vi "Link Test Channels.vi"(7 "gRPC ID in":T4, 8 "error in (no error)":errorcluster, 10 "Channels":T1[](array[typedef]), 11 "CIFCorePlugin in":refnum<class "CIFCorePlugin.lvclass">) -> (0 "error out":errorcluster, 3 "CIFCorePlugin out":refnum<class "CIFCorePlugin.lvclass">)   [LabVIEW 2021, in "CAN_Writer_NIXNET_Test_Helpers.lvlib"]
uses:
  CAN_Writer_NIXNET_Test_Helpers.lvlib
  <vilib>/CIF Foundation/CIF Core/CIFCore/Grpc/CIFCoreWrapper/CIFCoreWrapper.lvlib
  <vilib>/CIF Foundation/CIF Channels Core/ChannelCommon/ChannelCommon.lvlib
  <vilib>/CIF Foundation/CIF Channels Core/ChannelCommon/typedef/New FIFO Instance Configuration.ctl
  <vilib>/CIF Foundation/CIF Channels Core/CIFChannels/CIFChannels.lvclass
  <vilib>/CIF Foundation/CIF Core/CIFCore/Common/Typedef/FIFO Publisher.ctl
  <vilib>/CIF Foundation/CIF Core/CIFCore/Common/CIFCoreCommon.lvlib
  <vilib>/CIF Foundation/CIF Core/CIFCore/Grpc/CIFCoreChannel_client/RPC Messages/cif_channelcore_SetConnectionRequest.ctl
  <vilib>/CIF Foundation/CIF Core/CIFCore/Grpc/CIFCoreChannel_client/CIFCoreChannel_client.lvlib
  <vilib>/CIF Foundation/CIF Core/CIFCore/Class/CIFCorePlugin.lvclass
  <vilib>/gRPC/LabVIEW gRPC Library/Shared/grpcId.ctl
  <vilib>/gRPC/LabVIEW gRPC Library/grpc-lvsupport-release.lvlib
  <vilib>/CIF Foundation/CIF Core/CIFCore/Grpc/CIFCorePlugin_client/RPC Messages/cif_management_common_ChannelPattern.ctl
  <vilib>/CIF Foundation/CIF Core/CIFCore/Grpc/CIFCorePlugin_client/CIFCorePlugin_client.lvlib
  <vilib>/CIF Foundation/CIF Core/CIFCore/Grpc/CIFCorePlugin_client/RPC Messages/cif_management_common_ChannelDirection.ctl
  <vilib>/CIF Foundation/CIF Core/CIFCore/Grpc/CIFCorePlugin_client/RPC Messages/cif_management_common_Channel.ctl
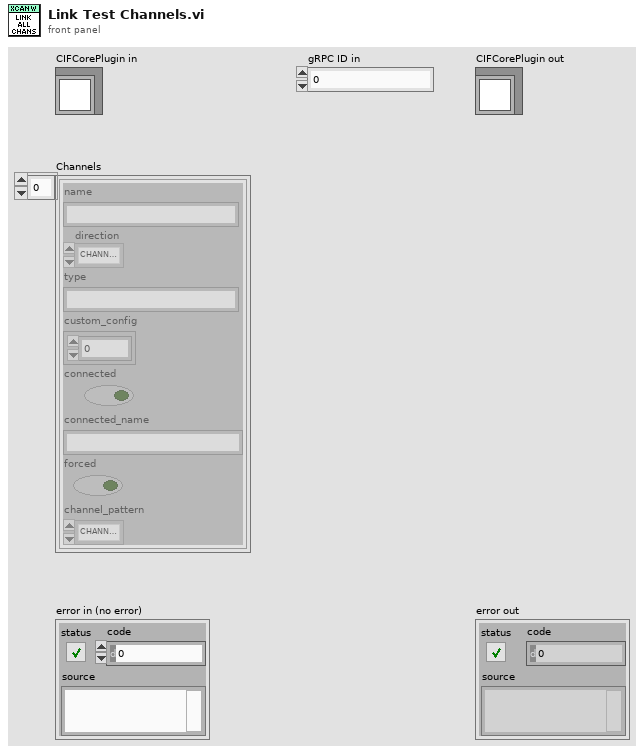
[diagram p1: front panel]
types:
  T1 = typedef "CIFCorePlugin_client.lvlib/cif_management_common_Channel.ctl" = cluster{"name":string, "direction":T2, "type":string, "custom_config":u8[], "connected":bool, "connected_name":string, "forced":bool, "channel_pattern":T3}
  T2 = typedef "CIFCorePlugin_client.lvlib/cif_management_common_ChannelDirection.ctl" = enum32{"CHANNELDIRECTION_UNKNOWN", "CHANNELDIRECTION_PUBLISHER", "CHANNELDIRECTION_SUBSCRIBER"}
  T3 = typedef "CIFCorePlugin_client.lvlib/cif_management_common_ChannelPattern.ctl" = enum32{"CHANNELPATTERN_UNKNOWN", "CHANNELPATTERN_TAG", "CHANNELPATTERN_FIFO", "CHANNELPATTERN_MULTIFIFO", "CHANNELPATTERN_BACKPRESSUREFIFO"}
  T4 = typedef "grpc-lvsupport-release.lvlib/grpcId.ctl" = u64
  T5 = typedef "ChannelCommon.lvlib/New FIFO Instance Configuration.ctl" = cluster{"Backpressure":bool, "Bytes/Message Override":u32, "Messages/FIFO Override":u32, "Custom Data":u8[]}
  T6 = typedef "CIFCoreCommon.lvlib/FIFO Publisher.ctl" = cluster{"Publisher Name":string, "New FIFO Instance Config":T5}
  T7 = typedef "CIFCoreChannel_client.lvlib/cif_channelcore_SetConnectionRequest.ctl" = cluster{"subscriber_name":string, "publisher_name":string, "custom_connect":u8[]}
  T8 = typedef "CIFChannels.lvclass/Direction.ctl" = enum16{"Publisher", "Subscriber"}
  T9 = typedef "ChannelCommon.lvlib/FIFO Config.ctl" = cluster{"Max Bytes/Msg":u64, "Max Msg/FIFO":u64, "Flags":u64, "Custom Data":u8[]}
  T10 = typedef "ChannelCommon.lvlib/FIFO Flags.ctl" = cluster{"Backpressure":bool}
  T11 = typedef "ChannelCommon.lvlib/New FIFO Instance Response.ctl" = cluster{"Publisher":string, "Custom Data":u8[]}
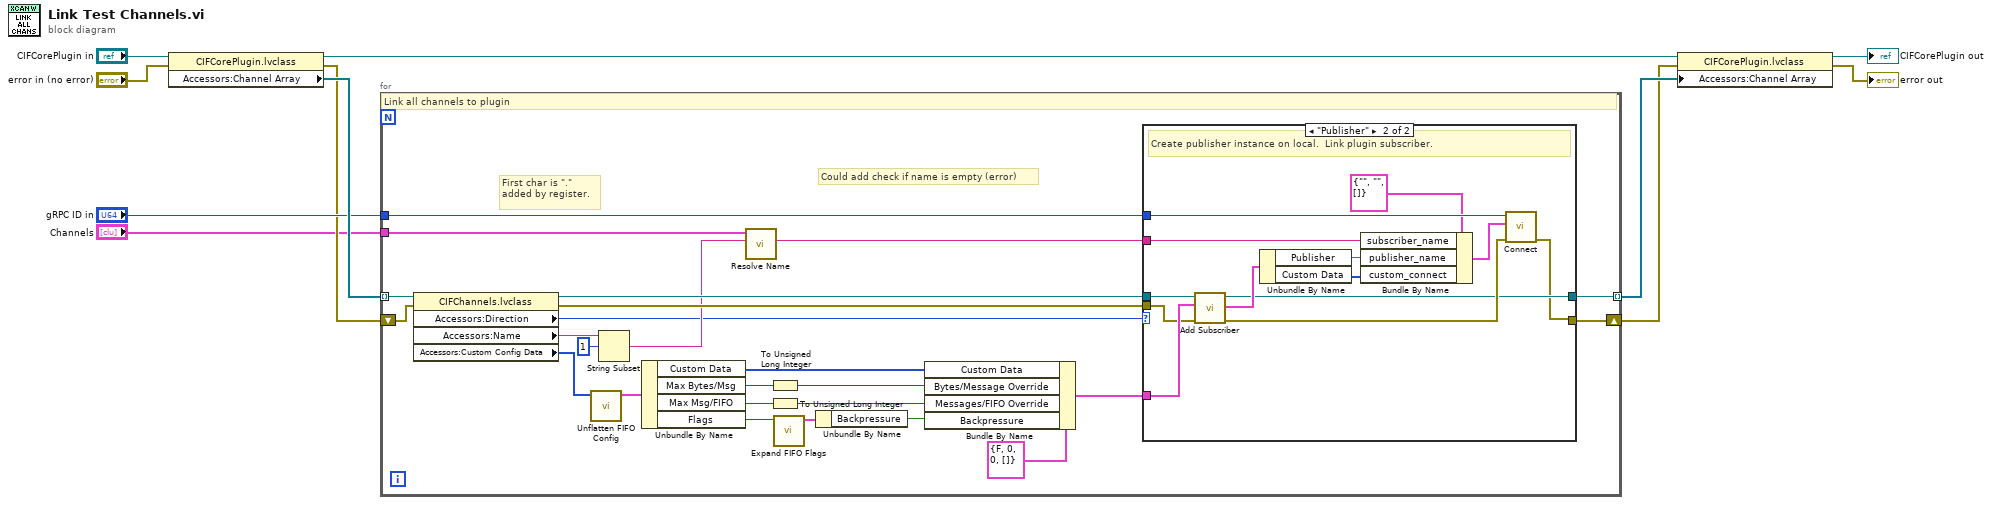
[diagram p0: block diagram]
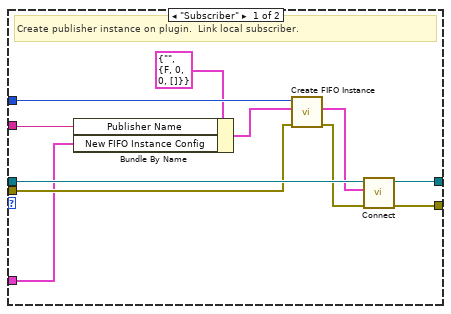
[diagram p2: hidden frame]
diagram:
  n1 = property class="CIFCorePlugin.lvclass"(reference="CIFCorePlugin in", error in="error in (no error)") -> (reference out=w6:refnum<class "CIFCorePlugin.lvclass">, error out=w7:errorcluster, "Accessors:Channel Array"=w10:refnum<class "CIFChannels.lvclass">[])
  n2 = for {
    tunnel: w10 -> [w36] mode=indexing
    tunnel: "gRPC ID in" -> [w33]
    tunnel: [w30] -> w5 mode=indexing
    shift-right: [w29] -> w3
    shift-left: w7 -> [w32]
    tunnel: "Channels" -> [w12]
    # "Could add check if name is empty (error)"
    # "First char is \".\" added by register."
    # "Link all channels to plugin"
    n3 = property class="CIFChannels.lvclass"(reference=w36, error in=w32) -> (reference out=w35:refnum<class "CIFChannels.lvclass">, error out=w31:errorcluster, "Accessors:Direction"=w17:T8, "Accessors:Name"=w15:string, "Accessors:Custom Config Data"=w34:u8[])
    n4 = call <vilib>:"Unflatten FIFO Config.vi"("Flattened Data in"=w34) -> ("FIFO Config out"=w28:T9)  [unwired: 9 in, 1 out]
    n5 = String Subset(string=w15, offset (0)=1) -> (substring=w18:string)  [unwired: 1 in]
    n6 = Unbundle By Name(w28) -> ("Custom Data"=w22:u8[], "Max Bytes/Msg"=w26:u64, "Max Msg/FIFO"=w25:u64, "Flags"=w27:u64)
    n7 = call <vilib>:"Resolve Name.vi"("Name in"=w18, "Channels"=w12) -> ("Name out"=w14:string)  [unwired: 7 in, 2 out]
    n8 = To Unsigned Long Integer(number=w26) -> (unsigned 32bit integer=w21:u32)
    n9 = To Unsigned Long Integer(number=w25) -> (unsigned 32bit integer=w20:u32)
    n10 = call <vilib>:"Expand FIFO Flags.vi"("FIFO Flags"=w27) -> ("Flags"=w24:T10)  [unwired: 10 in]
    n11 = Unbundle By Name(w24) -> ("Backpressure"=w23:bool)
    n12 = Bundle By Name(cluster=T5 {"Backpressure"=FALSE, "Bytes/Message Override"=0, "Messages/FIFO Override"=0, "Custom Data"=[]} ("New FIFO Instance Config"), "Custom Data"=w22, "Bytes/Message Override"=w21, "Messages/FIFO Override"=w20, "Backpressure"=w23) -> (w13:T5)
    n13 = case shown="\"Publisher\"" w17 {
      tunnel: w35 -> [w47 w60]
      tunnel: w33 -> [w46 w59]
      tunnel: w31 -> [w45 w53]
      tunnel: [w44 w51] -> w30
      tunnel: [w43 w50] -> w29
      tunnel: w13 -> [w38 w58]
      tunnel: w14 -> [w39 w49]
      frame "Subscriber" {
        # "Create publisher instance on plugin.  Link local subscriber."
        n14 = Bundle By Name(cluster=T6 {"Publisher Name"="", "New FIFO Instance Config"={"Backpressure"=FALSE, "Bytes/Message Override"=0, "Messages/FIFO Override"=0, "Custom Data"=[]}} ("New Publisher"), "Publisher Name"=w39, "New FIFO Instance Config"=w38) -> (w37:T6)
        n15 = call <vilib>:"Create FIFO Instance.vi"("error in"=w45, "New Publisher"=w37, "gRPC ID"=w46) -> ("error out"=w42:errorcluster, "FIFO Instance"=w41:T11)  [unwired: 6 in, 1 out]
        n16 = call-dynamic <vilib>:"Connect.vi"("error in (no error)"=w42, "Connection"=w41, "CIFChannels in"=w47) -> ("error out"=w43:errorcluster, "CIFChannels out"=w44:refnum<class "CIFChannels.lvclass">)  [unwired: 7 in]
      }
      frame "Publisher" {
        # "Create publisher instance on local.  Link plugin subscriber."
        n17 = call-dynamic "Add Subscriber.vi"("error in (no error)"=w53, "New FIFO Instance Config"=w58, "CIFChannels in"=w60) -> ("error out"=w52:errorcluster, "New FIFO Instance"=w57:T11, "CIFChannels out"=w51:refnum<class "CIFChannels.lvclass">)  [unwired: 6 in]
        n18 = Unbundle By Name(w57) -> ("Publisher"=w56:string, "Custom Data"=w55:u8[])
        n19 = Bundle By Name(cluster=T7 {"subscriber_name"="", "publisher_name"="", "custom_connect"=[]} ("Connection"), "subscriber_name"=w49, "publisher_name"=w56, "custom_connect"=w55) -> (w54:T7)
        n20 = call <vilib>:"Connect.vi"("error in"=w52, "Connection"=w54, "gRPC ID"=w59) -> ("error out"=w50:errorcluster)  [unwired: 7 in, 1 out]
      }
    }
  }
  n21 = property class="CIFCorePlugin.lvclass"(reference=w6, error in=w3, "Accessors:Channel Array"=w5) -> (reference out=→"CIFCorePlugin out":refnum<class "CIFCorePlugin.lvclass">, error out=→"error out":errorcluster)
